vi "Alertes.vi"() -> ()   [LabVIEW 2022 SP3]
uses:
  Variables globales/Variable glob Leybold.vi
  Variables globales/Variable glob Edwards.vi
  Variables globales/Variable glob Keller.vi
  Variables globales/Variable glob Th.vi
  Variables globales/Variable glob Pt.vi
  Variables globales/Variables glob EUROTHERM.vi
  Variables globales/Variable globale compteurs.vi
panel:
  out "sortie d'erreur":errorcluster
  out "ref au VI":refnum<vi>
  in  "OK":bool
  in  "Parametrer":bool
  in  "Alerte sur :":u16(ring) items=["Pressions EDWARDS ou LEYBOLD", "Min/Max Temperatures", "Ecart sur Temperatures", ""]
  # "definition des parametres\na surveiller"
  # "Ce logiciel et les informations qu'il contient, sont la propriété de l’IAS et ne peuvent être diffusés sans l’autorisation de la Station d’étalonnage"
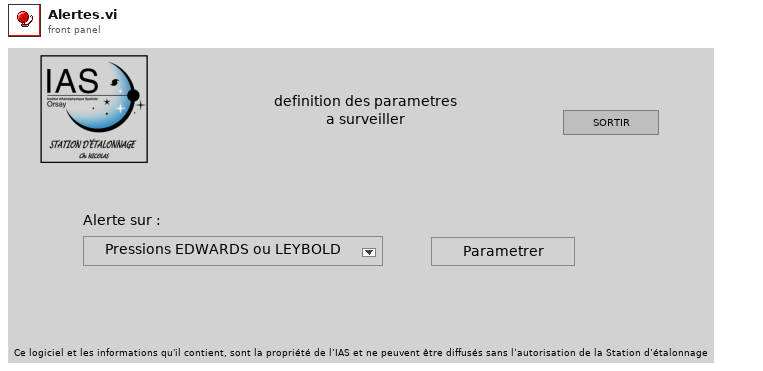
[diagram p1: front panel]
types:
  T1 = enum32{"Invalid", "Standard", "Closed", "Hidden", "Minimized", "Maximized"}
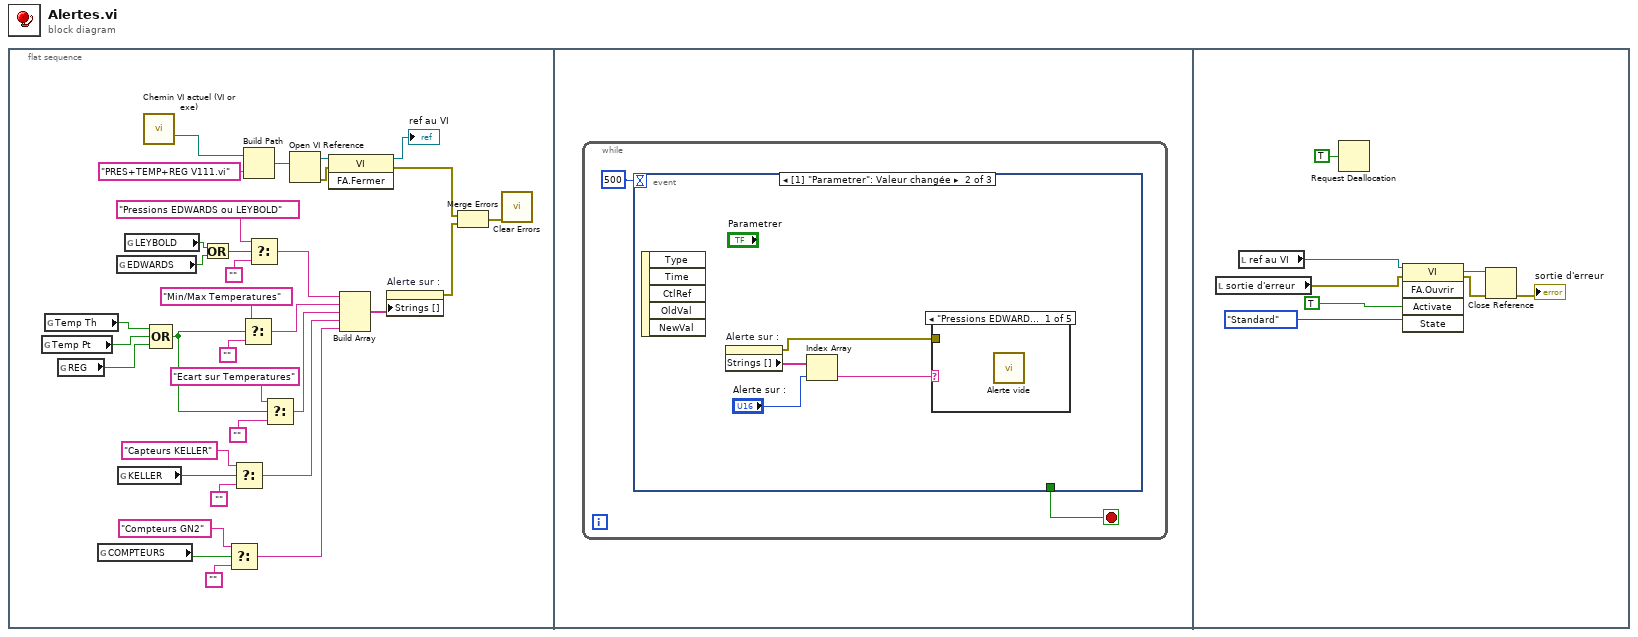
[diagram p0: block diagram]
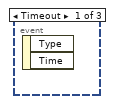
[diagram p2: hidden frame]
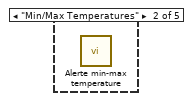
[diagram p3: hidden frame]
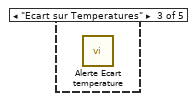
[diagram p4: hidden frame]
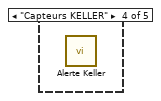
[diagram p5: hidden frame]
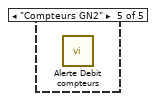
[diagram p6: hidden frame]
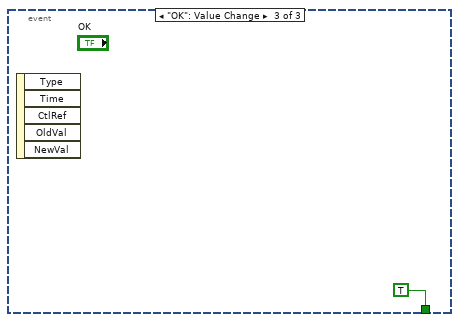
[diagram p7: hidden frame]
diagram:
  n1 = flat-sequence {
    frame #0 {
      n2 = global read "Variable glob Pt.vi" "Temp Pt"() -> (w8:bool)
      n3 = global read "Variable glob Th.vi" "Temp Th"() -> (w7:bool)
      n4 = global read "Variables glob EUROTHERM.vi" "REG"() -> (w9:bool)
      n5 = global read "Variable globale compteurs.vi" "COMPTEURS"() -> (w2:bool)
      n6 = global read "Variable glob Edwards.vi" "EDWARDS"() -> (w15:bool)
      n7 = global read "Variable glob Keller.vi" "KELLER"() -> (w22:bool)
      n8 = global read "Variable glob Leybold.vi" "LEYBOLD"() -> (w14:bool)
      n9 = call "Chemin VI actuel (VI or exe).vi"() -> ("VI or executable installation directory"=w5:path)  [unwired: 14 in, 1 out]
      n10 = Compound Arithmetic op=OR(w7, w8, w9) -> (w6:bool)
      n11 = Or(x=w14, y=w15) -> (x .or. y?=w16:bool)
      n12 = Select(t="Compteurs GN2" ("cas vrai"), s=w2, f="") -> (s? t:f=w1:string)
      n13 = Select(t="Capteurs KELLER" ("cas vrai"), s=w22, f="") -> (s? t:f=w28:string)
      n14 = Select(t="Min/Max Temperatures" ("cas vrai"), s=w6, f="") -> (s? t:f=w25:string)
      n15 = Build Path(base path=w5, name or relative path="PRES+TEMP+REG V111.vi" ("nom ou chemin relatif")) -> (appended path=w32:path)
      n16 = Select(t="Pressions EDWARDS ou LEYBOLD", s=w16, f="") -> (s? t:f=w24:string)
      n17 = Select(t="Ecart sur Temperatures" ("cas vrai"), s=w6, f="") -> (s? t:f=w29:string)
      n18 = Open VI Reference(vi path=w32) -> (vi reference=w33:refnum<vi>, error out=w34:errorcluster)  [unwired: 5 in]
      n19 = invoke class="VI" method="FA.Fermer"(reference=w33, error in=w34) -> (reference out=→"ref au VI":refnum<vi>, error out=w13:errorcluster)  [unwired: 1 in, 1 out]
      n20 = Build Array(w24, w25, w29, w28, w1) -> (w10:string[])
      n21 = property on="Alerte sur :" class="MDér (strict)"("Strings []"=w10) -> (error out=w12:errorcluster)  [unwired: 2 in, 1 out]
      n22 = Merge Errors(w13, w12) -> (w11:errorcluster)
      n23 = call <vilib>:"Clear Errors.vi"("error in (no error)"=w11) -> ()  [unwired: 5 in, 2 out]
    }
    frame #1 {
      n24 = while {
        stop <- w36 stop-if-true
        n25 = event shown="[1] \"Parametrer\": Valeur changée" {
          selector: _ -> [_ _ _]
          dyn-events: _ -> [_ _ _]
          timeout: 500 -> [_ _ _]
          tunnel: [_ _ TRUE] -> w36
          event Timeout {
            n26 = event-data() -> ()  [unwired: 1 in, 2 out]
          }
          event "Parametrer": Value Change {
            n27 = event-data() -> ()  [unwired: 1 in, 5 out]
            n28 = property on="Alerte sur :" class="MDér (strict)"() -> (error out=w37:errorcluster, "Strings []"=w40:string[])  [unwired: 2 in, 1 out]
            n29 = Index Array(array=w40, index="Alerte sur :") -> (element=w38:string)
            n30 = case shown="\"Pressions EDWARDS ou LEYBOLD\", Par défaut" w38 {
              tunnel: w37 -> [_ _ _ _ _]
              frame "Pressions EDWARDS ou LEYBOLD", Default {
                n31 = call "Alerte vide.vi"() -> ()  [unwired: 1 in]
              }
              frame "Min/Max Temperatures" {
                n32 = call "Alerte min-max temperature.vi"() -> ()  [unwired: 1 in]
              }
              frame "Ecart sur Temperatures" {
                n33 = call "Alerte Ecart temperature.vi"() -> ()  [unwired: 1 in]
              }
              frame "Capteurs KELLER" {
                n34 = call "Alerte Keller.vi"() -> ()  [unwired: 1 in]
              }
              frame "Compteurs GN2" {
                n35 = call "Alerte Debit compteurs.vi"() -> ()  [unwired: 1 in]
              }
            }
          }
          event "OK": Value Change {
            n36 = event-data() -> ()  [unwired: 1 in, 5 out]
          }
        }
      }
    }
    frame #2 {
      n37 = local read "sortie d'erreur"() -> (w49:errorcluster)
      n38 = local read "ref au VI"() -> (w48:refnum<vi>)
      n39 = Request Deallocation(TRUE ("flag")) -> ()
      n40 = invoke class="VI" method="FA.Ouvrir"(reference=w48, error in=w49, "Activate"=TRUE ("Activer ?"), "State"=T1."Standard" ("État")) -> (reference out=w46:refnum<vi>, error out=w47:errorcluster)  [unwired: 1 in, 3 out]
      n41 = Close Reference(reference=w46, error in (no error)=w47) -> (error out=→"sortie d'erreur":errorcluster)
    }
  }
